vi "MenuHandler.vi"(5 "tree control":refnum<vi>, 7 "main message queue":T1, 8 "error in":errorcluster, 9 "parameters":variant, 10 "menu string":string, 11 "NISE_CEF_Node in":refnum<class "NISE_CEF_Node.lvclass">) -> (0 "error out":errorcluster, 1 "refresh tree?":bool, 2 "Unhandled":bool, 3 "NISE_CEF_Node out":refnum<class "NISE_CEF_Node.lvclass">)   [LabVIEW 2014, in "NISE_CEF_Node.lvclass"]
uses:
  NISE_CEF_Node.lvclass
  <vilib>/NI/AMC/Message Queue.ctl
  <vilib>/NI/AMC/Message.ctl
  <vilib>/NI/Tools/Keyed Array/KeyedArray.ctl
  <vilib>/NI/Tools/Keyed Array/Tools_KeyedArray.lvlib
  <vilib>/NI/AMC/AMC.lvlib
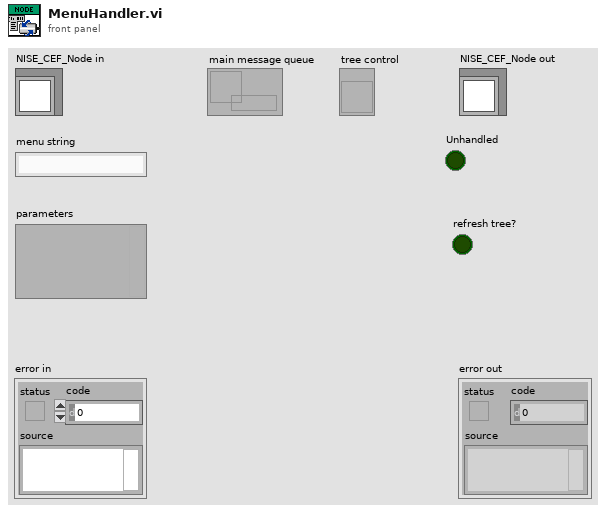
[diagram p1: front panel]
types:
  T1 = typedef "AMC.lvlib/Message Queue.ctl" = refnum<queue>
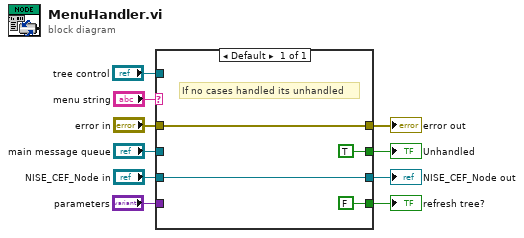
[diagram p0: block diagram]
diagram:
  n1 = case shown="Default" "menu string" {
    tunnel: [TRUE ("Unhandled")] -> w9
    tunnel: "parameters" -> [_]
    tunnel: "tree control" -> [_]
    tunnel: "main message queue" -> [_]
    tunnel: "NISE_CEF_Node in" -> [w13]
    tunnel: [w13] -> w4
    tunnel: [w12] -> w2
    tunnel: "error in" -> [w12]
    tunnel: [FALSE] -> w1
    frame Default {
      # "If no cases handled its unhandled"
    }
  }
  "error out" <- w2
  "NISE_CEF_Node out" <- w4
  "Unhandled" <- w9
  "refresh tree?" <- w1
